vi "Position Correction.vi"(7 "dP":dbl, 9 "Pos In":dbl, 10 "RevSpark Session":T1, 11 "Velocity In":dbl) -> (3 "Velocity Out":dbl)   [LabVIEW 2027]
uses:
  <vilib>/REV Custom Controls/REVSparkRefnum.ctl
  <resource>/objmgr/REVSpark.rc
  <vilib>/REVLibDriver/REVLibDriver.lvlib
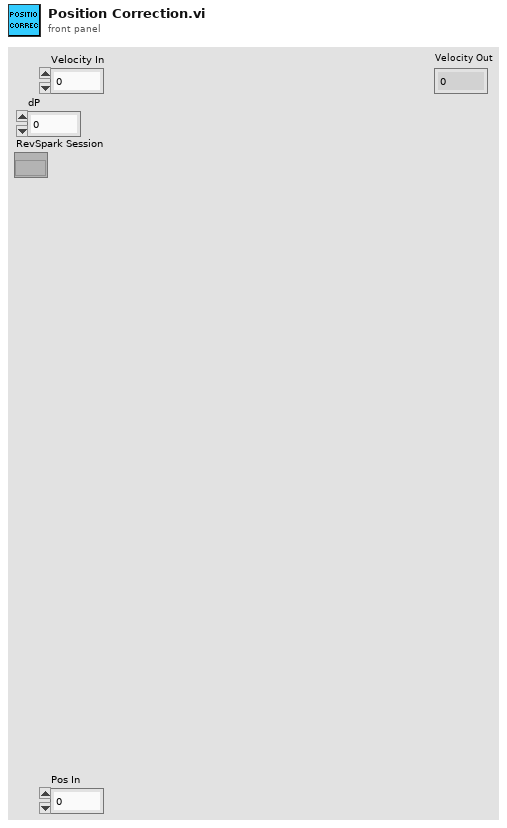
[diagram p1: front panel]
types:
  T1 = typedef "REVLibDriver.lvlib/REVSparkRefnum.ctl" = refnum<k20>
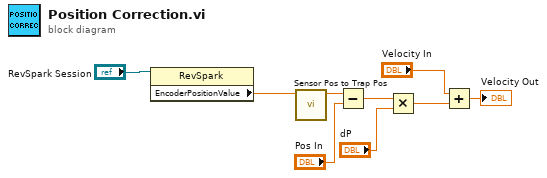
[diagram p0: block diagram]
diagram:
  n1 = property class="RevSpark"(reference="RevSpark Session") -> ("EncoderPositionValue"=w2:sgl)  [unwired: 1 in, 2 out]
  n2 = call "Sensor Pos to Trap Pos.vi"("Sensor Pos"=w2) -> ("Trapezoid Pos"=w5:dbl)  [unwired: 10 in]
  n3 = Subtract(x=w5, y="Pos In") -> (x-y=w4:dbl)
  n4 = Multiply(x=w4, y="dP") -> (x*y=w7:dbl)
  n5 = Add(x="Velocity In", y=w7) -> (x+y=→"Velocity Out":dbl)
